vi "Load.vi"(7 "Deck ID":string, 8 "error in (no error)":errorcluster, 9 "Message Queue":refnum<queue>, 10 "Path":path, 11 "Audio Data Reference":refnum<data-value>) -> (0 "error out":errorcluster)   [LabVIEW 2019, in "Audio File Input.lvlib"]
doc: "Sets up an asynchronous call to load the audio file given in Path."
uses:
  Audio File Input.lvlib
  Packed Libraries/Messaging.lvlibp/Message Cluster.ctl
  Packed Libraries/Messaging.lvlibp
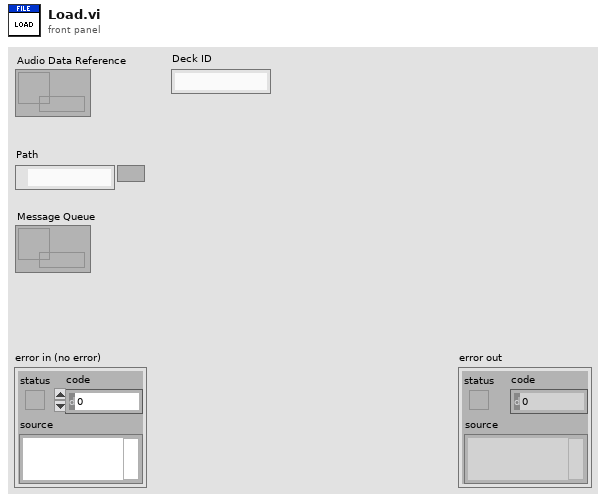
[diagram p1: front panel]
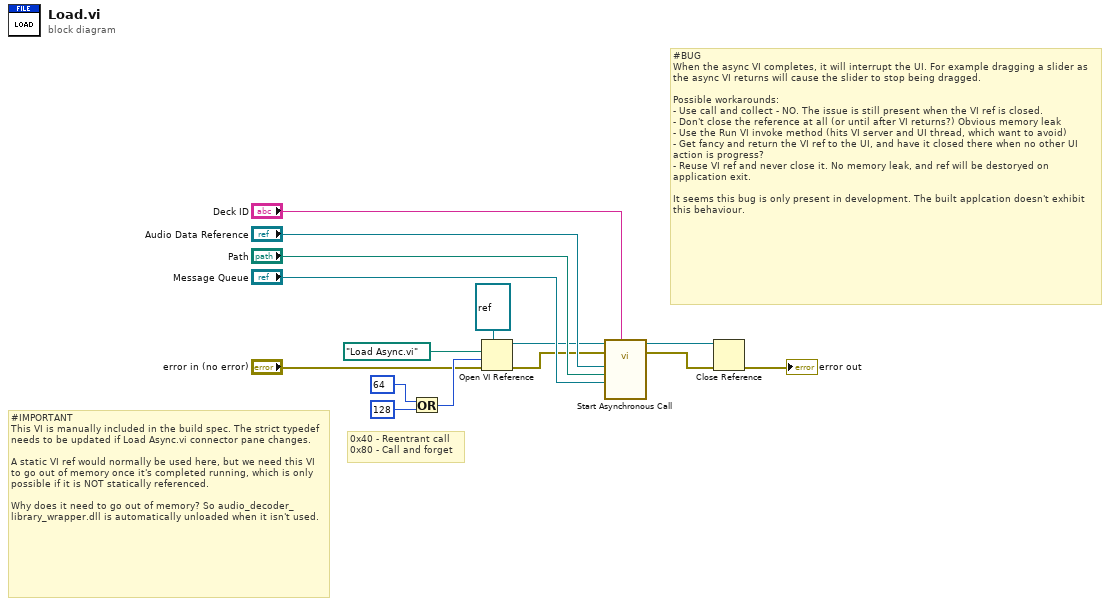
[diagram p0: block diagram]
diagram:
  # "#IMPORTANT\nThis VI is manually included in the build spec. The strict typedef needs to be updated if Load Async.vi connector pane changes.\n\nA static VI ref would normally be used here, but we need this VI to go out of memory once it's completed running, which is only possible if it is NOT statically referenced.\n\nWhy does it need to go out of memory? So audio_decoder_library_wrapper.dll is automatically unloaded when it isn't used."
  # "0x40 - Reentrant call\n0x80 - Call and forget"
  # "#BUG\nWhen the async VI completes, it will interrupt the UI. For example dragging a slider as the async VI returns will cause the slider to stop being dragged.\n\nPossible workarounds:\n- Use call and collect - NO. The issue is still present when the VI ref is closed.\n- Don't close the reference at all (or until after VI returns?) Obvious memory leak\n- Use the Run VI invoke method (hits VI server and UI thread, which want to avoid)\n- Get fancy and return the VI ref to the UI, and have it closed there when no other UI action is progress?\n- Reuse VI ref and never close it. No memory leak, and ref will be destoryed on application exit.\n\nIt seems this bug is only present in development. The built applcation doesn't exhibit this behaviour."
  n1 = Or(x=64 ("options"), y=128 ("options")) -> (x .or. y?=w4:i32)
  n2 = Open VI Reference(type specifier VI Refnum (for type only)=refnum<vi> refnum, vi path=path "Load Async.vi", options=w4, error in (no error)="error in (no error)") -> (vi reference=w10:refnum<vi>, error out=w9:errorcluster)  [unwired: 2 in]
  n3 = call-by-ref "Start Asynchronous Call"(reference=w10, error in=w9, "Deck ID"="Deck ID", "Message Queue"="Message Queue", "Path"="Path", "Audio Data Reference"="Audio Data Reference") -> (reference out=w7:refnum<vi>, error out=w8:errorcluster)  [unwired: 7 in, 1 out]
  n4 = Close Reference(reference=w7, error in (no error)=w8) -> (error out=→"error out":errorcluster)
